vi "sr_golden.vi"() -> ()   [LabVIEW 2020]
panel:
  out "Out1":dbl
  in  "Num1":dbl
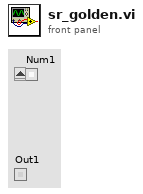
[diagram p1: front panel]
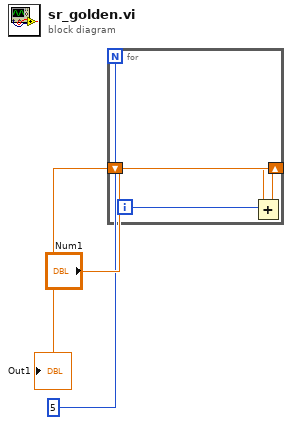
[diagram p0: block diagram]
diagram:
  n1 = for "L1" {
    N: 5 ("N5") -> [_]
    shift-right: [w4] -> w2
    shift-left: "Num1" -> [w6]
    i -> [w5]
    n2 = Add ("A1")(x=w6, y=w5) -> (x+y=w4:dbl)
  }
  "Out1" <- w2
